vi "to string.vi"(8 "error in":errorcluster, 11 "Modbus Slave configuration in":refnum<class "Modbus Module configuration.lvclass">) -> (0 "error out":errorcluster, 1 "data":string, 2 "version":string, 3 "Modbus Slave configuration out":refnum<class "Modbus Module configuration.lvclass">)   [LabVIEW 2015, in "Modbus Module configuration.lvclass"]
doc: "Provides an interface for saving a module configuration to a file or other serialized data source. It is recommended that all children of this class store data in two sets--data required for its own initialization, and any data required for parent initialization--and that each implementation uses the <b>Call Parent Method</b> primitive to serialize parent information.Platypus Framework 1.0.1.65\nNI Systems Engineering - National Instruments"
uses:
  Modbus Module configuration.lvclass
  Modbus Module configuration.lvclass/Modbus Module configuration.ctl
  <vilib>/NI/Tag Bus Module Framework/module configuration/TBM module configuration.lvclass
  module channel/Modbus Module Channel.lvclass
  <vilib>/NI/Configuration Framework/serializable configuration/NISE_CEF_serializable configuration.lvclass
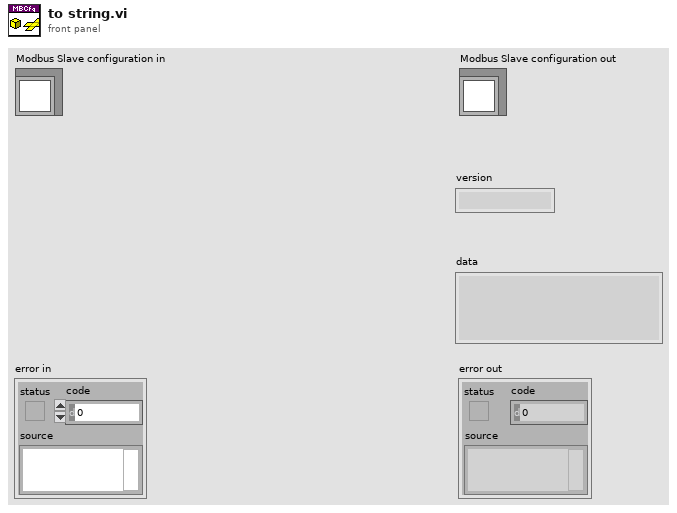
[diagram p1: front panel]
types:
  T1 = typedef "Modbus Module configuration.lvclass/modbus class.ctl" = enum16{"TCP master", "TCP slave", "serial master", "serial slave"}
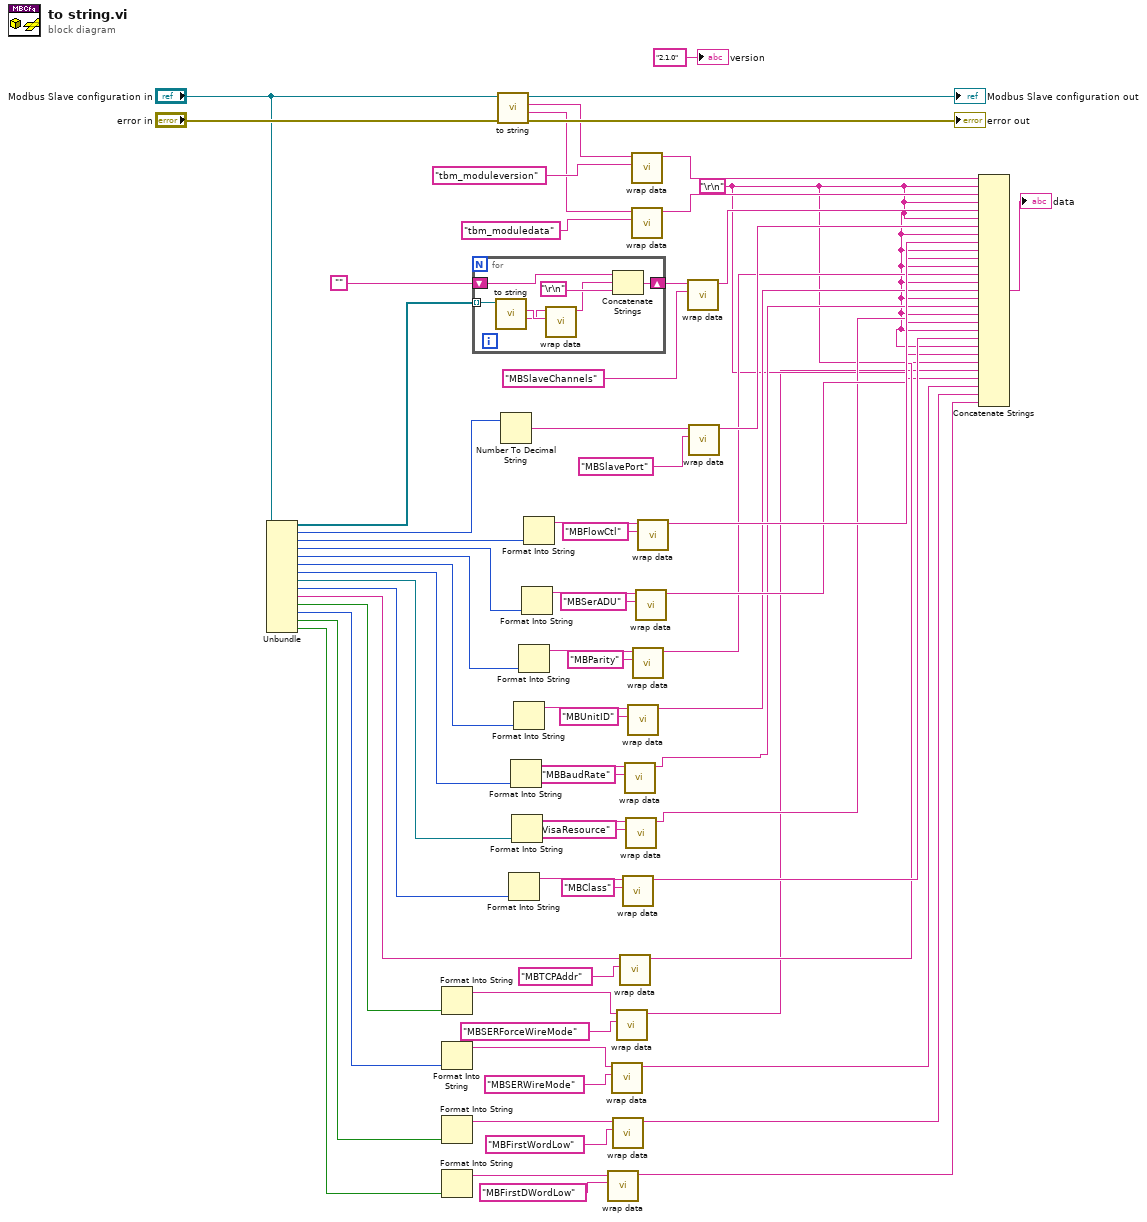
[diagram p0: block diagram]
diagram:
  w11 = "\r\n"
  n1 = Unbundle("Modbus Slave configuration in") -> (w56:refnum<class "Modbus Module Channel.lvclass">[], w51:u16, w47:u16, w33:enum16{"RTU", "ASCII"}, w32:u16, w31:u8, w30:u32, w29:refnum<visa-resource-name>, w28:T1, w20:string, w14:bool, w15:i16, w8:bool, w5:bool)
  n2 = Format Into String(w14) -> (resulting string=w13:string)  [unwired: 3 in, 1 out]
  n3 = Format Into String(w15) -> (resulting string=w12:string)  [unwired: 3 in, 1 out]
  n4 = Format Into String(w8) -> (resulting string=w3:string)  [unwired: 3 in, 1 out]
  n5 = Format Into String(w5) -> (resulting string=w4:string)  [unwired: 3 in, 1 out]
  n6 = for {
    tunnel: w56 -> [w72] mode=indexing
    shift-right: [w75] -> w54
    shift-left: "" -> [w74]
    n7 = call-dynamic "to string.vi"("channel in"=w72) -> ("channel data"=w70:string, "identifier"=w71:string)  [unwired: 7 in, 2 out]
    n8 = call <vilib>:"wrap data.vi"("identifier"=w71, "data to wrap"=w70) -> ("wrapped data"=w73:string)  [unwired: 9 in]
    n9 = Concatenate Strings(w74, w73, "\r\n") -> (w75:string)
  }
  n10 = call-parent "to string.vi"("error in"="error in", "module configuration in"="Modbus Slave configuration in") -> ("error out"=→"error out":errorcluster, "data"=w61:string, "version"=w62:string, "module configuration out"=→"Modbus Slave configuration out":refnum<class "Modbus Module configuration.lvclass">)  [unwired: 6 in]
  n11 = Number To Decimal String(number=w51) -> (decimal integer string=w50:string)  [unwired: 1 in]
  n12 = Format Into String(w28) -> (resulting string=w35:string)  [unwired: 3 in, 1 out]
  n13 = Format Into String(w30) -> (resulting string=w40:string)  [unwired: 3 in, 1 out]
  n14 = Format Into String(w29) -> (resulting string=w36:string)  [unwired: 3 in, 1 out]
  n15 = Format Into String(w31) -> (resulting string=w39:string)  [unwired: 3 in, 1 out]
  n16 = Format Into String(w32) -> (resulting string=w43:string)  [unwired: 3 in, 1 out]
  n17 = Format Into String(w33) -> (resulting string=w44:string)  [unwired: 3 in, 1 out]
  n18 = Format Into String(w47) -> (resulting string=w48:string)  [unwired: 3 in, 1 out]
  n19 = call <vilib>:"wrap data.vi"("identifier"="MBFirstDWordLow", "data to wrap"=w4) -> ("wrapped data"=w1:string)  [unwired: 9 in]
  n20 = call <vilib>:"wrap data.vi"("identifier"="MBSERWireMode", "data to wrap"=w12) -> ("wrapped data"=w9:string)  [unwired: 9 in]
  n21 = call <vilib>:"wrap data.vi"("identifier"="MBFirstWordLow", "data to wrap"=w3) -> ("wrapped data"=w2:string)  [unwired: 9 in]
  n22 = call <vilib>:"wrap data.vi"("identifier"="MBSERForceWireMode", "data to wrap"=w13) -> ("wrapped data"=w10:string)  [unwired: 9 in]
  n23 = call <vilib>:"wrap data.vi"("identifier"="MBTCPAddr", "data to wrap"=w20) -> ("wrapped data"=w19:string)  [unwired: 9 in]
  n24 = call <vilib>:"wrap data.vi"("identifier"="MBClass", "data to wrap"=w35) -> ("wrapped data"=w21:string)  [unwired: 9 in]
  n25 = call <vilib>:"wrap data.vi"("identifier"="MBBaudRate", "data to wrap"=w40) -> ("wrapped data"=w23:string)  [unwired: 9 in]
  n26 = call <vilib>:"wrap data.vi"("identifier"="MBVisaResource", "data to wrap"=w36) -> ("wrapped data"=w22:string)  [unwired: 9 in]
  n27 = call <vilib>:"wrap data.vi"("identifier"="MBUnitID", "data to wrap"=w39) -> ("wrapped data"=w24:string)  [unwired: 9 in]
  n28 = call <vilib>:"wrap data.vi"("identifier"="tbm_moduleversion" ("additional identifier"), "data to wrap"=w62) -> ("wrapped data"=w64:string)  [unwired: 9 in]
  n29 = call <vilib>:"wrap data.vi"("identifier"="tbm_moduledata" ("additional identifier"), "data to wrap"=w61) -> ("wrapped data"=w63:string)  [unwired: 9 in]
  n30 = call <vilib>:"wrap data.vi"("identifier"="MBParity", "data to wrap"=w43) -> ("wrapped data"=w25:string)  [unwired: 9 in]
  n31 = call <vilib>:"wrap data.vi"("identifier"="MBSerADU", "data to wrap"=w44) -> ("wrapped data"=w26:string)  [unwired: 9 in]
  n32 = call <vilib>:"wrap data.vi"("identifier"="MBFlowCtl", "data to wrap"=w48) -> ("wrapped data"=w27:string)  [unwired: 9 in]
  n33 = call <vilib>:"wrap data.vi"("identifier"="MBSlaveChannels" ("additional identifier"), "data to wrap"=w54) -> ("wrapped data"=w58:string)  [unwired: 9 in]
  n34 = call <vilib>:"wrap data.vi"("identifier"="MBSlavePort" ("additional identifier"), "data to wrap"=w50) -> ("wrapped data"=w52:string)  [unwired: 9 in]
  n35 = Concatenate Strings(w64, w11, w63, w11, w58, w11, w52, w11, w27, w11, w26, w11, w25, w11, w24, w11, w23, w11, w22, w11, w21, w11, w19, w11, w10, w11, w9, w2, w1) -> (→"data":string)
  "version" <- "2.1.0" ("current version")
